vi "Dequeue Data.vi"(8 "error in":errorcluster, 11 "UI GUID":string) -> (0 "error out":errorcluster, 3 "Data":string[][](array[string]))   [LabVIEW 2025, in "CAN-LIN Raw Bus Capture UI.lvlib"]
uses:
  CAN-LIN Raw Bus Capture UI.lvlib
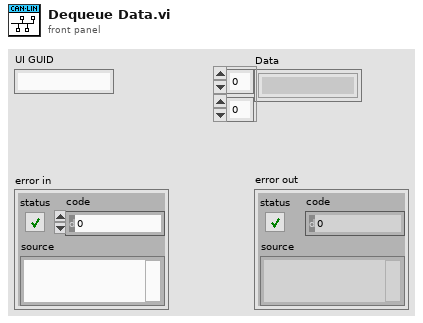
[diagram p1: front panel]
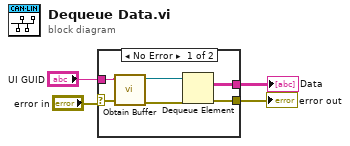
[diagram p0: block diagram]
diagram:
  n1 = case shown="No Error" "error in" {
    selector: "error in" -> [w8 w11]
    tunnel: [w10 w11] -> w3
    tunnel: [w6 _] -> w2
    tunnel: "UI GUID" -> [w5 _]
    frame No Error {
      n2 = call "Obtain Buffer.vi"("error in (no error)"=w8, "UI GUID"=w5) -> ("error out"=w9:errorcluster, "Table Queue"=w7:refnum<queue>)  [unwired: 8 in]
      n3 = Dequeue Element(queue=w7, error in (no error)=w9) -> (element=w6:string[][], error out=w10:errorcluster)  [unwired: 1 in, 2 out]
    }
    frame Error {
    }
  }
  "Data" <- w2
  "error out" <- w3
